vi "Exec Write Probe.vi"() -> ()   [LabVIEW 2026]
doc: "Probe: which VI execution properties VI Server can WRITE. Each write is on its own error chain; the errors come back as an array in the order of the writes."
panel:
  out "error out":errorcluster
  out "write errors":errorcluster[](array[cluster])
  in  "vi path":path
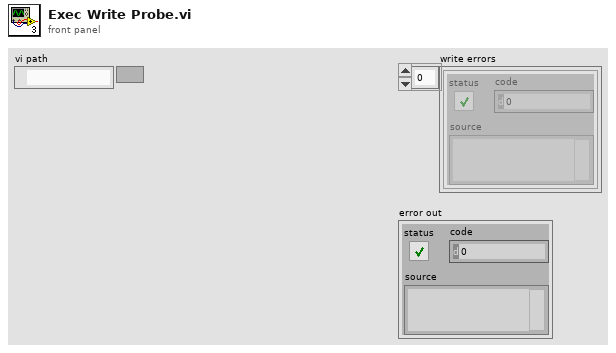
[diagram p1: front panel]
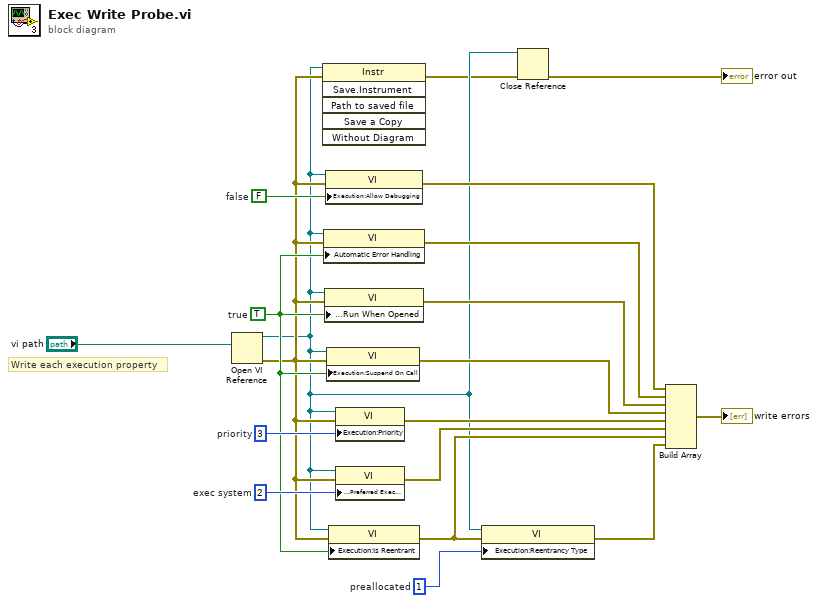
[diagram p0: block diagram]
diagram:
  w14 = u32 1  # preallocated
  w16 = 2  # exec system
  w17 = u16 3  # priority
  w15 = TRUE  # true
  w18 = FALSE  # false
  # "Write each execution property"
  n1 = Open VI Reference(vi path="vi path") -> (vi reference=w4:refnum<vi>, error out=w5:errorcluster)  [unwired: 5 in]
  n2 = invoke class="Instr" method="Save.Instrument"(reference=w4, error in=w5) -> (error out=w3:errorcluster)  [unwired: 4 in, 5 out]
  n3 = property class="VI"(reference=w4, error in=w5, "Automatic Error Handling"=w15) -> (error out=w12:errorcluster)  [unwired: 1 out]
  n4 = property class="VI"(reference=w4, error in=w5, "Execution:Run When Opened"=w15) -> (error out=w11:errorcluster)  [unwired: 1 out]
  n5 = property class="VI"(reference=w4, error in=w5, "Execution:Allow Debugging"=w18) -> (error out=w13:errorcluster)  [unwired: 1 out]
  n6 = property class="VI"(reference=w4, error in=w5, "Execution:Suspend On Call"=w15) -> (error out=w10:errorcluster)  [unwired: 1 out]
  n7 = property class="VI"(reference=w4, error in=w5, "Execution:Is Reentrant"=w15) -> (error out=w7:errorcluster)  [unwired: 1 out]
  n8 = property class="VI"(reference=w4, error in=w5, "Execution:Priority"=w17) -> (error out=w9:errorcluster)  [unwired: 1 out]
  n9 = property class="VI"(reference=w4, error in=w5, "Execution:Preferred Exec System"=w16) -> (error out=w8:errorcluster)  [unwired: 1 out]
  n10 = property class="VI"(reference=w4, error in=w7, "Execution:Reentrancy Type"=w14) -> (error out=w6:errorcluster)  [unwired: 1 out]
  n11 = Close Reference(reference=w4, error in (no error)=w3) -> (error out=→"error out":errorcluster)
  n12 = Build Array(w13, w12, w11, w10, w9, w8, w7, w6) -> (→"write errors":errorcluster[])
